vi "ADI_IMU_ADIS16448_Loop.vi"(8 "error in":errorcluster, 11 "ADI_IMU_DevRef":T1={"ADI IMU DevRef"={"DevStatus"={"status"=FALSE, "code"=0, "source"=""}, "Handle"=0, "SPI Bus"=enum."SPI On-Board, CS0", "Device Found"=FALSE, "Device Ready"=FALSE, "Yaw Axis"=enum."Z", "AHRS Algorithm"=enum."Complementary", "Serial"=0, "Lot ID 2"=0, "Lot ID 1"=0, "Product ID"=0}, "InterruptRef"={"DevStatus"={"status"=FALSE, "code"=0, "source"=""}, "InterruptIndex"=enum."0"}}) -> (0 "error out":errorcluster, 1 "Device Found":bool)   [LabVIEW 2016, in "ADIS16448_IMU.lvlib"]
doc: "Periodically reads the ADI MXP IMU valuse and makes data available for use elsewhere in your robot project. Place this block within PeriodicTasks.vi outside any loops."
uses:
  ADIS16448_IMU.lvlib
  ADI_IMU_ADIS16448_InterruptDevRef.ctl
  ADI_IMU_ADIS16448_IMUDevRef.ctl
  <vilib>/Rock Robotics/SystemInterfaces/spilib/spi_bus.ctl
  <vilib>/Rock Robotics/WPI/Interrupt/WPI_InterruptRef.ctl
  <vilib>/Rock Robotics/SystemInterfaces/Interrupt/FPGA_InterruptIndex.ctl
  <vilib>/Rock Robotics/WPI/SPI/WPI_SPIDevRef.ctl
  ADI_IMU_ADIS16448_Registers.ctl
  <vilib>/Platform/TimedLoop/XDataNode/timing_clust.ctl
  <vilib>/Platform/TimedLoop/XDataNode/nitl_modes.ctl
  <vilib>/Platform/TimedLoop/XDataNode/wakeup.ctl
  <vilib>/Rock Robotics/SystemInterfaces/Utilities/FPGA_UtilitiesRead LocalTime.vi
  <vilib>/Rock Robotics/SystemInterfaces/Interrupt/FPGA_WaitOnInterrupt.vi
  <vilib>/Rock Robotics/WPI/Utilities/WPI_UtilitiesTimebaseConstants.vi
  <vilib>/Rock Robotics/SystemInterfaces/Interrupt/FPGA_InterruptReadTimestamp.vi
  <vilib>/Platform/TimedLoop/XDataNode/XDataNode.xnode
  <vilib>/Platform/TimedLoop/XDataNode/XDNodeRunTimeDep.lvlib
  <vilib>/ptbypt/NI_PtbyPt.lvlib
panel:
  in  "Main Name":string
  out "SPS":dbl
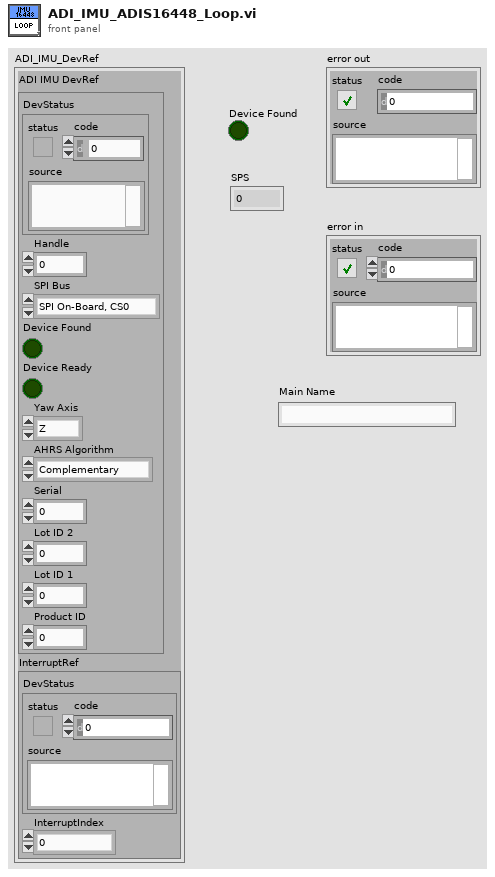
[diagram p1: front panel]
types:
  T1 = typedef "ADIS16448_IMU.lvlib/ADI_IMU_ADIS16448_InterruptDevRef.ctl" = cluster{"ADI IMU DevRef":T2, "InterruptRef":T4}
  T2 = typedef "ADIS16448_IMU.lvlib/ADI_IMU_ADIS16448_IMUDevRef.ctl" = cluster{"DevStatus":errorcluster, "Handle":i32, "SPI Bus":T3, "Device Found":bool, "Device Ready":bool, "Yaw Axis":enum16{"X", "Y", "Z"}, "AHRS Algorithm":enum16{"Complementary", "Madgwick"}, "Serial":u16, "Lot ID 2":u16, "Lot ID 1":u16, "Product ID":u16}
  T3 = typedef "spi_bus.ctl" = enum16{"SPI On-Board, CS0", "SPI On-Board, CS1", "SPI On-Board, CS2", "SPI On-Board, CS3", "SPI MXP", "Invalid"}
  T4 = typedef "WPI_InterruptRef.ctl" = cluster{"DevStatus":errorcluster, "InterruptIndex":T5}
  T5 = typedef "FPGA_InterruptIndex.ctl" = enum8{"0", "1", "2", "3", "4", "5", "6", "7", "Invalid"}
  T6 = typedef "WPI_SPIDevRef.ctl" = cluster{"DevStatus":errorcluster, "Handle":i32, "SPI Bus":T3}
  T7 = cluster{"read mode":enum16{"polling", "blocking"}, "write mode":enum16{"polling", "blocking"}}
  T8 = cluster{"X Angle":dbl, "Y Angle":dbl, "Z Angle":dbl}
  T9 = enum32{"Bad", "Idle", "Run top level", "Running"}
  T10 = typedef "XDNodeRunTimeDep.lvlib/timing_clust.ctl" = cluster{"Expected End [f-1]":u64, "Actual End [f-1]":u64, "Finished Late? [f-1]":bool, "Expected End [i-1]":u64, "Actual End [i-1]":u64, "Finished Late? [i-1]":bool, "Expected Start [i]":u64, "Actual Start [i]":u64, "Expected Start [f]":u64, "Actual Start [f]":u64, "Source Name":string, "Structure Name":string, "Period":i64, "Deadline":i64, "Offset":i64, "Start":i64, "Priority":i32, "Timeout":i32, "Mode":T11, "Wakeup Reason":T12, "Error":errorcluster, "Source Type":string, "Secondary Source Type":string, "Global End Time":u64, "Global Start Time":u64, "Frame Duration":u64, "Iteration Duration":u64, "Assigned CPU":i32, "I/O Scan Engine Mode":u32}
  T11 = typedef "XDNodeRunTimeDep.lvlib/nitl_modes.ctl" = enum32{"No Change", "Process missed periods, maintain original phase", "Discard missed periods, maintain original phase", "Process missed periods, ignore original phase", "Discard missed periods, ignore original phase"}
  T12 = typedef "XDNodeRunTimeDep.lvlib/wakeup.ctl" = enum32{"Normal", "Aborted", "Asynchronous wakeup", "Timing source error", "Timed loop error", "Timeout"}
  T13 = cluster{"X Gyro":dbl, "Y Gyro":dbl, "Z Gyro":dbl, "X Accel":dbl, "Y Accel":dbl, "Z Accel":dbl, "X Mag":dbl, "Y Mag":dbl, "Z Mag":dbl, "Pressure":dbl, "Temp":dbl}
  T14 = typedef "ADIS16448_IMU.lvlib/ADI_IMU_ADIS16448_Registers.ctl" = u8
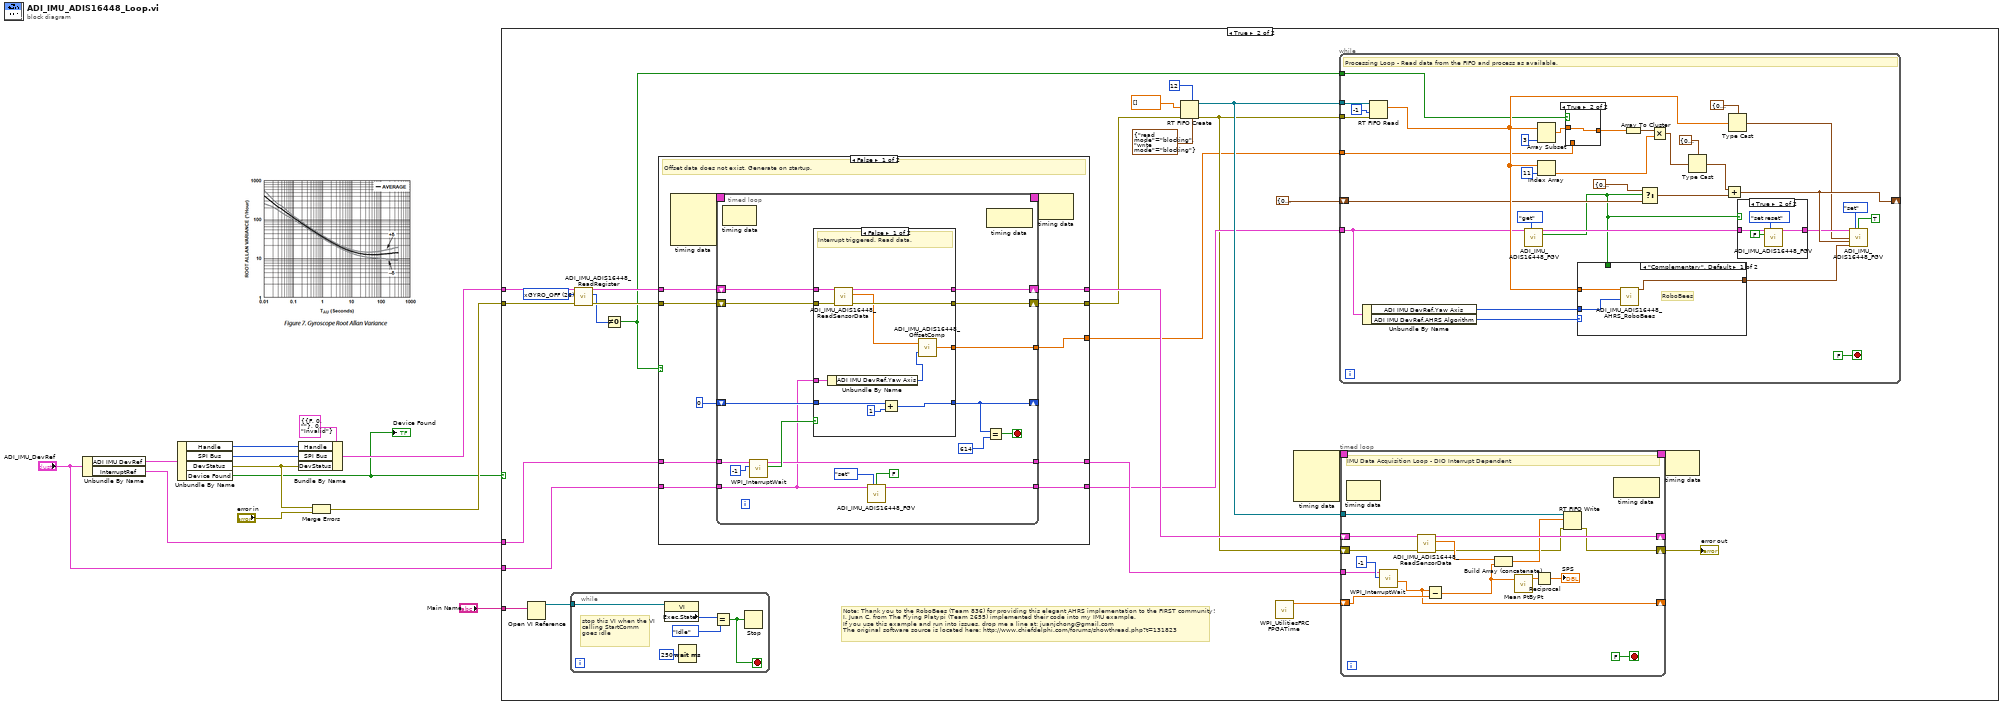
[diagram p0: block diagram]
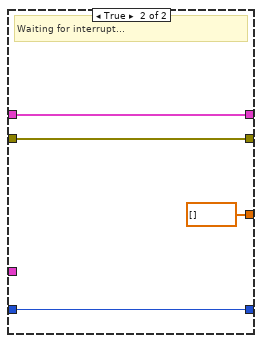
[diagram p3: hidden frame]
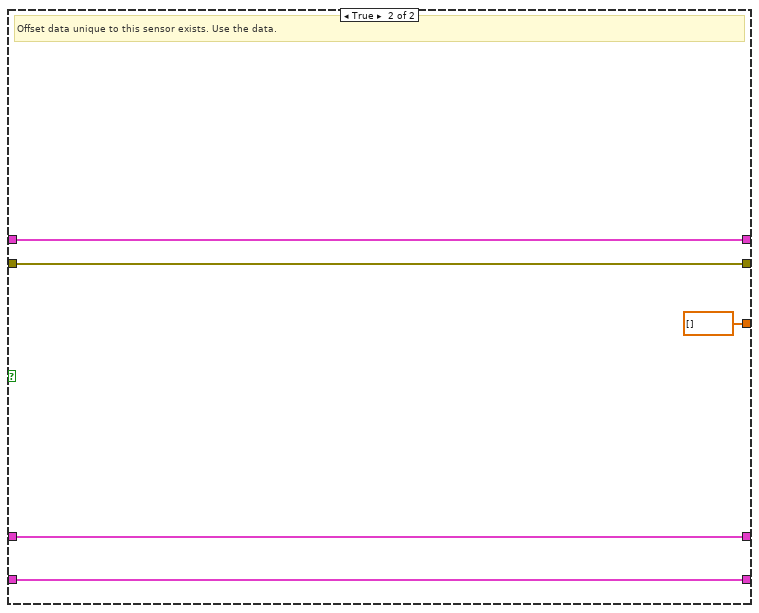
[diagram p4: hidden frame]
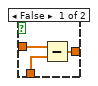
[diagram p5: hidden frame]
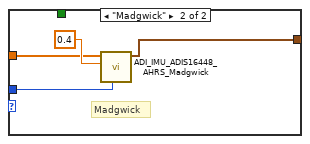
[diagram p6: hidden frame]
diagram:
  n1 = Unbundle By Name("ADI_IMU_DevRef") -> ("ADI IMU DevRef"=w8:T2, "InterruptRef"=w4:T4)
  n2 = Unbundle By Name(w8) -> ("Handle"=w11:i32, "SPI Bus"=w10:T3, "DevStatus"=w9:errorcluster, "Device Found"=w2:bool)
  "Device Found" <- w2
  n3 = Bundle By Name(cluster=T6 {"DevStatus"={"status"=FALSE, "code"=0, "source"=""}, "Handle"=0, "SPI Bus"=enum."Invalid"} ("SPIDevRef out"), "Handle"=w11, "SPI Bus"=w10, "DevStatus"=w9) -> (w6:T6)
  n4 = Merge Errors(w9, "error in") -> (w5:errorcluster)
  n5 = case shown="True" w2 {
    tunnel: w6 -> [_ w24]
    tunnel: w5 -> [_ w23]
    tunnel: w4 -> [_ w34]
    tunnel: "ADI_IMU_DevRef" -> [_ w33]
    tunnel: "Main Name" -> [_ w13]
    frame False {
    }
    frame True {
      w20 = T14 26 items=["zGYRO_OFF"=30, "yGYRO_OFF"=28, "xGYRO_OFF"=26, "GLOB_CMD"=62, "SEQ_CNT"=58, "SMPL_PRD"=54, "SENS_AVG"=56, "MSC_CTRL"=52, "zACCEL_OFF"=36, "yACCEL_OFF"=34, "xACCEL_OFF"=32, "ERROR_FLAGS"=60, "TEMP"=24, "BARO"=22, "Z_MAG"=20, "Y_MAG"=18, "X_MAG"=16, "Z_ACCEL"=14, "Y_ACCEL"=12, "X_ACCEL"=10, "Z_GYRO"=8, "Y_GYRO"=6, "X_GYRO"=4, "PROD_ID"=86, "LOT_ID2"=84, "LOT_ID1"=82, "SERIAL_NUM"=88] ("ADIS16448 Register")
      # "Note: Thank you to the RoboBees (Team 836) for providing this elegant AHRS implementation to the FIRST community!\nI, Juan C. from The Flying Platypi (Team 2655) implemented their code into my IMU example.\nIf you use this example and run into issues, drop me a line at: juanjchong@gmail.com\nThe original software source is located here: http://www.chiefdelphi.com/forums/showthread.php?t=131823"
      n6 = Open VI Reference(vi path=w13) -> (vi reference=w14:refnum<vi>)  [unwired: 1 in, 5 out]
      n7 = while {
        tunnel: w14 -> [w40]
        stop <- w39 stop-if-true
        # "stop this VI when the VI calling StartComm goes idle"
        n8 = property class="VI"(reference=w40) -> ("Exec.State"=w42:T9)  [unwired: 1 in, 2 out]
        n9 = Wait (ms)(milliseconds to wait=u32 250) -> ()  [unwired: 1 out]
        n10 = Equal?(x=w42, y=T9."Idle" ("Execution:State")) -> (x = y?=w39:bool)
        n11 = Stop(stop? (T)=w39) -> ()
      }
      n12 = call "ADI_IMU_ADIS16448_ReadRegister.vi"("error in (no error)"=w23, "ADIS16448 Register"=w20, "SPIDevRef in"=w24) -> ("error out"=w21:errorcluster, "Register Value"=w19:u16, "SPIDevRef out"=w22:T6)  [unwired: 6 in]
      n13 = Not Equal To 0?(x=w19) -> (x != 0?=w18:bool)
      n14 = case shown="False" w18 {
        tunnel: w22 -> [w72 w116]
        tunnel: w21 -> [w71 w115]
        tunnel: [w70 w116] -> w35
        tunnel: w34 -> [w69 w114]
        tunnel: w33 -> [w68 w113]
        tunnel: [w67 w114] -> w32
        tunnel: [w66 w113] -> w31
        tunnel: [w65 w115] -> w30
        tunnel: [w64 dbl[] [] ("Offset Compensated Data")] -> w25
        frame False {
          # "Offset data does not exist. Generate on startup."
          n15 = node-c288() -> (w75:T10)  [unwired: 4 in]
          n16 = timed-loop {
            shift-right: [w91] -> w70
            shift-left: w72 -> [w87]
            shift-right: [w92] -> w65
            shift-left: w71 -> [w86]
            shift-right: [w83] -> _
            shift-left: 0 -> [w90]
            timing: w75 -> [_]
            timing-out: [_] -> w74
            tunnel: [w77] -> w64
            tunnel: w69 -> [w81]
            tunnel: [w80] -> w67
            tunnel: w68 -> [w76]
            tunnel: [w79] -> w66
            stop <- w82 stop-if-true
            n17 = node-c288() -> ()  [unwired: 1 in, 1 out]
            n18 = call <vilib>:"WPI_InterruptWait.vi"("Timeout (ms)"=-1, "InterruptRef"=w81) -> ("Timed Out"=w88:bool, "InterruptRef"=w80:T4)  [unwired: 5 in, 3 out]
            n19 = case shown="False" w88 {
              tunnel: [w105 w107] -> w92
              tunnel: [w104 w108] -> w91
              tunnel: w86 -> [w103 w107]
              tunnel: w87 -> [w102 w108]
              tunnel: w90 -> [w99 w109]
              tunnel: [w101 w109] -> w83
              tunnel: [w97 dbl[] [] ("Offset Compensated Data")] -> w77
              tunnel: w76 -> [w96 _]
              frame False {
                # "Interrupt triggered. Read data."
                n20 = Unbundle By Name(w96) -> ("ADI IMU DevRef.Yaw Axis"=w95:enum16{"X", "Y", "Z"})
                n21 = call "ADI_IMU_ADIS16448_ReadSensorData.vi"("error in (no error)"=w103, "SPIDevRef in"=w102) -> ("error out"=w105:errorcluster, "Data Array"=w98:dbl[], "SPIDevRef out"=w104:T6)  [unwired: 7 in]
                n22 = Add(x=w99, y=1) -> (x+y=w101:i32)
                n23 = call "ADI_IMU_ADIS16448_OffsetComp.vi"("Yaw Axis"=w95, "Raw Data"=w98) -> ("Offset Compensated Data"=w97:dbl[])
              }
              frame True {
                # "Waiting for interrupt..."
              }
            }
            n24 = call "ADI_IMU_ADIS16448_FGV.vi"("ADI IMU Interrupt DevRef"=w76, "Operation"=enum16{"set", "get", "set reset"}."set", "Sensor Ready?"=FALSE) -> ("ADI IMU Interrupt DevRef Out"=w79:T1)  [unwired: 6 in, 6 out]
            n25 = node-c288() -> ()  [unwired: 1 in, 1 out]
            n26 = Equal?(x=w83, y=614) -> (x = y?=w82:bool)
          }
          n27 = node-c288(w74) -> ()  [unwired: 1 out]
        }
        frame True {
          # "Offset data unique to this sensor exists. Use the data."
        }
      }
      n28 = RT FIFO Create(1:dbl[] [] ("appended array"), 3:w30, 6:u32 12 ("elements in array (1)"), 7:T7 {"read mode"=enum."blocking", "write mode"=enum."blocking"} ("r/w modes (polling,polling)")) -> (8:w38:refnum<k33>, 11:w29:errorcluster)  [unwired: 4 in, 1 out]
      n29 = call <vilib>:"WPI_UtilitiesFRC FPGATime.vi"() -> ("FPGA Time"=w17:dbl)  [unwired: 10 in, 1 out]
      n30 = node-c288() -> (w16:T10)  [unwired: 4 in]
      n31 = while {
        tunnel: w38 -> [w147]
        shift-right: [w143] -> _
        shift-left: T8 {"X Angle"=0.0, "Y Angle"=0.0, "Z Angle"=0.0} ("IMU Angles") -> [w144]
        tunnel: w25 -> [w139]
        tunnel: w29 -> [w146]
        tunnel: w18 -> [w117]
        tunnel: w31 -> [w140]
        stop <- FALSE stop-if-true
        # "Processing Loop - Read data from the FIFO and process as available."
        n32 = Unbundle By Name(w140) -> ("ADI IMU DevRef.Yaw Axis"=w142:enum16{"X", "Y", "Z"}, "ADI IMU DevRef.AHRS Algorithm"=w141:enum16{"Complementary", "Madgwick"})
        n33 = RT FIFO Read(0:w147, 2:-1 ("timeout in ms (0)"), 3:w146) -> (9:w145:dbl[])  [unwired: 1 in, 4 out]
        n34 = call "ADI_IMU_ADIS16448_FGV.vi"("ADI IMU Interrupt DevRef"=w140, "Operation"=enum16{"set", "get", "set reset"}."get") -> ("ADI IMU Interrupt DevRef Out"=w124:T1, "Reset Out"=w119:bool)  [unwired: 7 in, 5 out]
        n35 = Array Subset(array=w145, length=3) -> (w136:dbl[])  [unwired: 1 in]
        n36 = Index Array(array=w145, index=11) -> (element=w123:dbl)
        n37 = case shown="True" w117 {
          tunnel: w139 -> [w151 _]
          tunnel: w136 -> [w150 w152]
          tunnel: [w149 w152] -> w135
          frame False {
            n38 = Subtract(x=w150, y=w151) -> (x-y=w149:dbl[])
          }
          frame True {
          }
        }
        n39 = case shown="\"Complementary\", Default" w141 {
          tunnel: w145 -> [w155 w158]
          tunnel: w142 -> [w154 w157]
          tunnel: w119 -> [_ _]
          tunnel: [w153 w156] -> w118
          frame "Complementary", Default {
            # "RoboBees"
            n40 = call "ADI_IMU_ADIS16448_AHRS_RoboBees.vi"("Yaw Axis"=w154, "IMU Rates"=w155) -> ("Output"=w153:cluster{"Pitch":dbl, "Roll":dbl, "Yaw":dbl})  [unwired: 5 in, 3 out]
          }
          frame "Madgwick" {
            # "Madgwick"
            n41 = call "ADI_IMU_ADIS16448_AHRS_Madgwick.vi"("Yaw Axis"=w157, "Beta"=0.4, "Data"=w158) -> ("Output"=w156:cluster{"Pitch":dbl, "Roll":dbl, "Yaw":dbl})  [unwired: 8 in]
          }
        }
        n42 = Array To Cluster(array=w135) -> (cluster=w134:cluster{"[0]":dbl, "[1]":dbl, "[2]":dbl})
        n43 = Select(t=T8 {"X Angle"=0.0, "Y Angle"=0.0, "Z Angle"=0.0} ("IMU Angles"), s=w119, f=w144) -> (s? t:f=w132:T8)
        n44 = Multiply(x=w134, y=w123) -> (x*y=w127:cluster{"[0]":dbl, "[1]":dbl, "[2]":dbl})
        n45 = Type Cast(type=T8 {"X Angle"=0.0, "Y Angle"=0.0, "Z Angle"=0.0} ("IMU Angles"), x=w127) -> (*(type *) &x=w128:T8)
        n46 = Add(x=w128, y=w132) -> (x+y=w143:T8)
        n47 = Type Cast(type=T13 {"X Gyro"=0.0, "Y Gyro"=0.0, "Z Gyro"=0.0, "X Accel"=0.0, "Y Accel"=0.0, "Z Accel"=0.0, "X Mag"=0.0, "Y Mag"=0.0, "Z Mag"=0.0, "Pressure"=0.0, "Temp"=0.0} ("IMU Data"), x=w145) -> (*(type *) &x=w121:T13)
        n48 = case shown="True" w119 {
          tunnel: [w160 w163] -> w125
          tunnel: w124 -> [w160 w162]
          frame False {
          }
          frame True {
            n49 = call "ADI_IMU_ADIS16448_FGV.vi"("ADI IMU Interrupt DevRef"=w162, "Operation"=enum16{"set", "get", "set reset"}."set reset", "Reset"=FALSE) -> ("ADI IMU Interrupt DevRef Out"=w163:T1)  [unwired: 6 in, 6 out]
          }
        }
        n50 = call "ADI_IMU_ADIS16448_FGV.vi"("ADI IMU Interrupt DevRef"=w125, "Operation"=enum16{"set", "get", "set reset"}."set", "Sensor Ready?"=TRUE, "IMU Data"=w121, "IMU Angles"=w143, "IMU AHRS"=w118) -> ()  [unwired: 3 in, 7 out]
      }
      n51 = timed-loop {
        tunnel: w38 -> [w58]
        shift-right: [w54] -> _
        shift-left: w35 -> [w56]
        shift-right: [w53] -> w28
        shift-left: w29 -> [w55]
        tunnel: w32 -> [w52]
        shift-right: [w50] -> _
        shift-left: w17 -> [w51]
        timing: w16 -> [_]
        timing-out: [_] -> w15
        stop <- FALSE stop-if-true
        # "IMU Data Acquisition Loop - DIO Interrupt Dependent"
        n52 = node-c288() -> ()  [unwired: 1 in, 1 out]
        n53 = call <vilib>:"WPI_InterruptWait.vi"("Timeout (ms)"=-1, "InterruptRef"=w52) -> ("TimeStamp"=w50:dbl)  [unwired: 5 in, 4 out]
        n54 = call "ADI_IMU_ADIS16448_ReadSensorData.vi"("error in (no error)"=w55, "SPIDevRef in"=w56) -> ("error out"=w47:errorcluster, "Data Array"=w49:dbl[], "SPIDevRef out"=w54:T6)  [unwired: 7 in]
        n55 = Subtract(x=w50, y=w51) -> (x-y=w46:dbl)
        n56 = Build Array (concatenate)(w49, w46) -> (w48:dbl[])
        n57 = call <vilib>:"Mean PtByPt.vi"("x"=w46) -> ("mean"=w45:dbl)  [unwired: 3 in, 1 out]
        n58 = Reciprocal(x=w45) -> (1/x=→"SPS":dbl)
        n59 = RT FIFO Write(0:w58, 1:w48, 3:w47) -> (11:w53:errorcluster)  [unwired: 2 in, 3 out]
        n60 = node-c288() -> ()  [unwired: 1 in, 1 out]
      }
      "error out" <- w28
      n61 = node-c288(w15) -> ()  [unwired: 1 out]
    }
  }
